vi "Create Handle Messages Method.vi"(8 "error in (no error)":errorcluster, 11 "Process Generator in":refnum<class "Process Generator.lvclass">) -> (0 "error out":errorcluster, 3 "Process Generator out":refnum<class "Process Generator.lvclass">)   [LabVIEW 2020, in "Process Generation.lvlib" / "Process Generator.lvclass"]
uses:
  Process Generator.lvclass
  <vilib>/Utility/traverseref.llb/TRef TravTarget.ctl
  Process Generator.lvclass/Process Generator.ctl
  Support/Support.lvlib
  <vilib>/Utility/traverseref.llb/VI Scripting - Traverse.lvlib
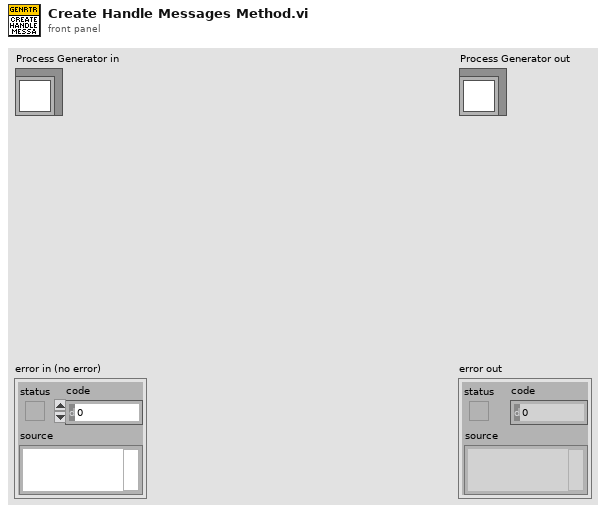
[diagram p1: front panel]
types:
  T1 = typedef "TRef TravTarget.ctl" = enum16{"FP", "BD", "Other"}
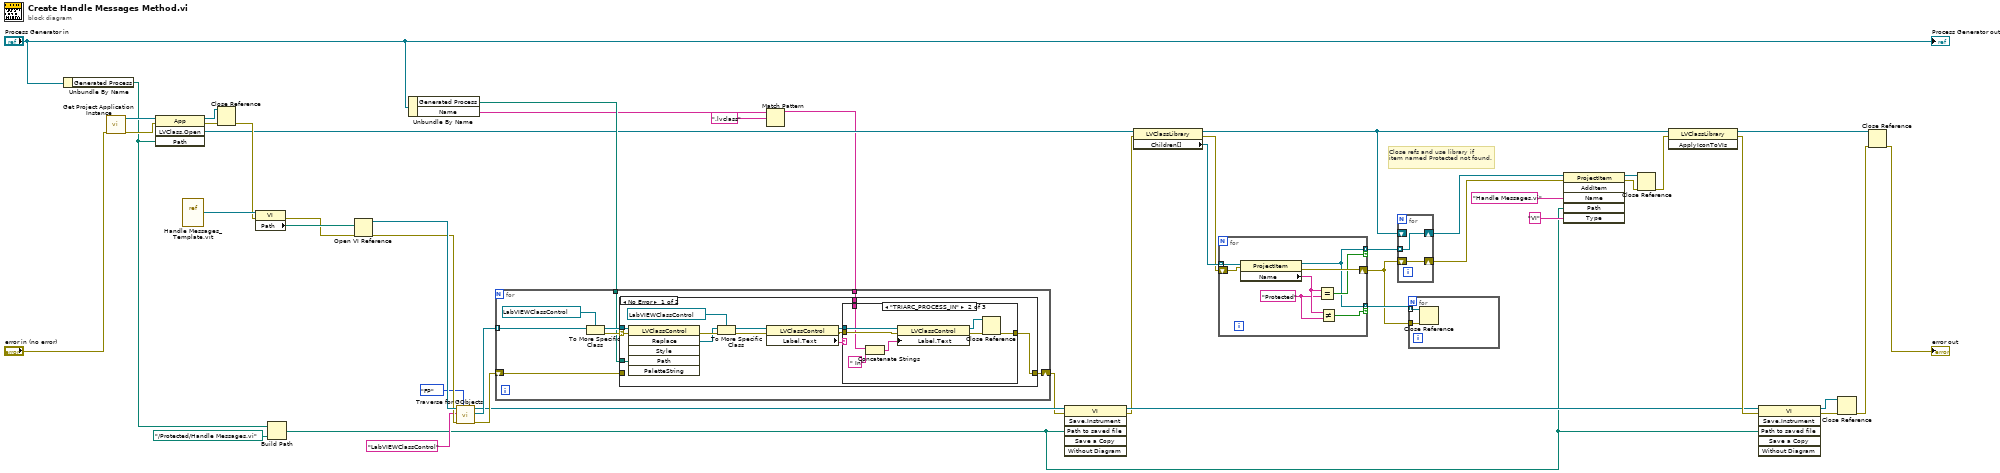
[diagram p0: block diagram]
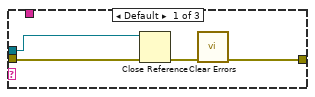
[diagram p2: hidden frame]
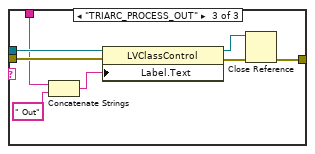
[diagram p3: hidden frame]
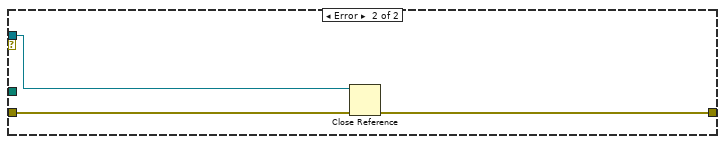
[diagram p4: hidden frame]
diagram:
  # "Close refs and use library if \nitem named Protected not found."
  n1 = Unbundle By Name("Process Generator in") -> ("Generated Process"=w44:path)
  n2 = call "Get Project Application Instance.vi"("error in (no error)"="error in (no error)") -> ("error out"=w46:errorcluster, "Application out"=w47:refnum<vi>)  [unwired: 9 in]
  n3 = invoke class="App" method="LVClass.Open"(reference=w47, error in=w46, "Path"=w44) -> (reference out=w25:refnum<vi>, error out=w36:errorcluster, "LVClass.Open"=w23:refnum<vi>)  [unwired: 1 in, 1 out]
  n4 = vi-ref "Handle Messages_Template.vit"() -> (w45:refnum<vi>)
  n5 = Close Reference(reference=w25, error in (no error)=w36) -> (error out=w26:errorcluster)
  n6 = property class="VI"(reference=w45, error in=w26) -> (error out=w35:errorcluster, "Path"=w38:path)  [unwired: 1 out]
  n7 = Build Path(base path=w44, name or relative path=path "../Protected/Handle Messages.vi") -> (appended path=w2:path)
  n8 = Open VI Reference(vi path=w38, error in (no error)=w35) -> (vi reference=w39:refnum<vi>, error out=w34:errorcluster)  [unwired: 4 in]
  n9 = Unbundle By Name("Process Generator in") -> ("Generated Process"=w27:path, "Name"=w13:string)
  n10 = call <vilib>:"Traverse for GObjects.vi"("Traverse Target"=TRef_TravTarget."FP", "error in (no error)"=w34, "Class Name"="LabVIEWClassControl", "VI Refnum"=w39) -> ("error out"=w28:errorcluster, "References"=w29:refnum<vi>[], "dup VI Refnum"=w5:refnum<vi>)  [unwired: 4 in, 1 out]
  n11 = Match Pattern(string=w13, regular expression=".lvclass") -> (before substring=w12:string)  [unwired: 1 in, 3 out]
  n12 = for {
    tunnel: w29 -> [w55] mode=indexing
    tunnel: w27 -> [w51]
    shift-right: [w50] -> w3
    shift-left: w28 -> [w49]
    tunnel: w12 -> [w48]
    n13 = To More Specific Class(target class=refnum<vi> refnum ("reference out"), reference=w55) -> (specific class reference=w52:refnum<vi>, error out=w53:errorcluster)  [unwired: 1 in]
    n14 = case shown="No Error" w53 {
      selector: w53 -> [w68 _]
      tunnel: w52 -> [w67 w89]
      tunnel: w51 -> [w66 _]
      tunnel: [w65 w90] -> w50
      tunnel: w49 -> [_ w91]
      tunnel: w48 -> [w62 _]
      frame No Error {
        n15 = invoke on="Invoke Node" class="LVClassControl" method="Replace"(reference=w67, error in=w68, "Path"=w66) -> (error out=w64:errorcluster, "Replace"=w59:refnum<vi>)  [unwired: 3 in, 4 out]
        n16 = To More Specific Class(target class=refnum<vi> refnum ("reference out"), reference=w59, error in=w64) -> (specific class reference=w58:refnum<vi>, error out=w57:errorcluster)
        n17 = property class="LVClassControl"(reference=w58, error in=w57) -> (reference out=w61:refnum<vi>, error out=w60:errorcluster, "Label.Text"=w63:string)
        n18 = case shown="\"TRIARC_PROCESS_IN\"" w63 {
          tunnel: [w70 w74 w82] -> w65
          tunnel: w61 -> [w72 w79 w87]
          tunnel: w60 -> [w69 w78 w86]
          tunnel: w62 -> [_ w77 w85]
          frame Default {
            n19 = Close Reference(reference=w72, error in (no error)=w69) -> (error out=w71:errorcluster)
            n20 = call <vilib>:"Clear Errors.vi"("error in (no error)"=w71) -> ("error out"=w70:errorcluster)  [unwired: 5 in, 1 out]
          }
          frame "TRIARC_PROCESS_IN" {
            n21 = Concatenate Strings(w77, " In" ("string")) -> (w75:string)
            n22 = property class="LVClassControl"(reference=w79, error in=w78, "Label.Text"=w75) -> (reference out=w73:refnum<vi>, error out=w80:errorcluster)
            n23 = Close Reference(reference=w73, error in (no error)=w80) -> (error out=w74:errorcluster)
          }
          frame "TRIARC_PROCESS_OUT" {
            n24 = Concatenate Strings(w85, " Out" ("string")) -> (w83:string)
            n25 = property class="LVClassControl"(reference=w87, error in=w86, "Label.Text"=w83) -> (reference out=w81:refnum<vi>, error out=w88:errorcluster)
            n26 = Close Reference(reference=w81, error in (no error)=w88) -> (error out=w82:errorcluster)
          }
        }
      }
      frame Error {
        n27 = Close Reference(reference=w89, error in (no error)=w91) -> (error out=w90:errorcluster)
      }
    }
  }
  n28 = invoke on="Invoke Node" class="VI" method="Save.Instrument"(reference=w5, error in=w3, "Path to saved file"=w2) -> (reference out=w4:refnum<vi>, error out=w1:errorcluster)  [unwired: 3 in, 4 out]
  n29 = property class="LVClassLibrary"(reference=w23, error in=w1) -> (reference out=w15:refnum<vi>, error out=w21:errorcluster, "Children[]"=w22:refnum<vi>[])
  n30 = for {
    tunnel: w22 -> [w99] mode=indexing
    tunnel: [w95] -> w19 mode=indexing if=w96
    shift-right: [w98] -> w18
    shift-left: w21 -> [w97]
    tunnel: [w95] -> w20 mode=indexing if=w92
    w93 = "Protected"
    n31 = property class="ProjectItem"(reference=w99, error in=w97) -> (reference out=w95:refnum<vi>, error out=w98:errorcluster, "Name"=w94:string)
    n32 = Equal?(x=w94, y=w93) -> (x = y?=w96:bool)
    n33 = Not Equal?(x=w94, y=w93) -> (x != y?=w92:bool)
  }
  n34 = for {
    tunnel: w19 -> [w101] mode=indexing
    shift-right: [w101] -> w16
    shift-left: w15 -> [_]
    shift-right: [w100] -> w17
    shift-left: w18 -> [w100]
  }
  n35 = for {
    tunnel: w20 -> [w103] mode=indexing
    tunnel: w18 -> [w102]
    n36 = Close Reference(reference=w103, error in (no error)=w102) -> ()  [unwired: 1 out]
  }
  n37 = invoke class="ProjectItem" method="AddItem"(reference=w16, error in=w17, "Name"="Handle Messages.vi", "Path"=w2, "Type"="VI") -> (reference out=w41:refnum<vi>, error out=w42:errorcluster)  [unwired: 1 in, 4 out]
  n38 = Close Reference(reference=w41, error in (no error)=w42) -> (error out=w8:errorcluster)
  n39 = invoke class="LVClassLibrary" method="ApplyIconToVIs"(reference=w15, error in=w8) -> (reference out=w10:refnum<vi>, error out=w7:errorcluster)  [unwired: 1 in, 1 out]
  n40 = invoke on="Invoke Node" class="VI" method="Save.Instrument"(reference=w4, error in=w7, "Path to saved file"=w2) -> (reference out=w31:refnum<vi>, error out=w32:errorcluster)  [unwired: 3 in, 4 out]
  n41 = Close Reference(reference=w31, error in (no error)=w32) -> (error out=w6:errorcluster)
  n42 = Close Reference(reference=w10, error in (no error)=w6) -> (error out=→"error out":errorcluster)
  "Process Generator out" <- "Process Generator in"
